vi "[ce low] Eval y=f(x).vi"(4 "include end point":bool, 5 "# points":u32=100, 6 "vm cmd":T1(ring), 7 "VC Handle":T2=-1, 8 "error in":errorcluster, 9 "formula info":cluster{"formula":string, "x-variable":string}={"formula"="", "x-variable"="t"}, 10 "end":dbl=1.0 format="%.2f", 11 "start":dbl format="%.2f") -> (0 "error out":errorcluster, 1 "dx":dbl format="%.2f", 2 "f(x)":dbl[](array[numeric]) format="%.2f", 3 "x":dbl[](array[numeric]) format="%.2f")   [LabVIEW 2021]
doc: "::: CalcExpress Toolkit :::\nCopyright (c) 2000-2026 Konstantin Shifershteyn. All rights reserved."
uses:
  cetypes.llb/VarMan Variable Context Handle.ctl
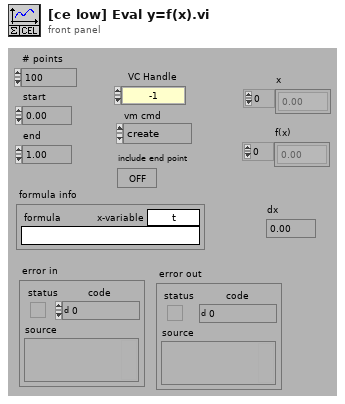
[diagram p1: front panel]
types:
  T1 = enum16{"create", "destroy", "set value", "get value"}
  T2 = typedef "VarMan Variable Context Handle.ctl" = i32
  T3 = typedef "VarMan Error Code.ctl" = u16
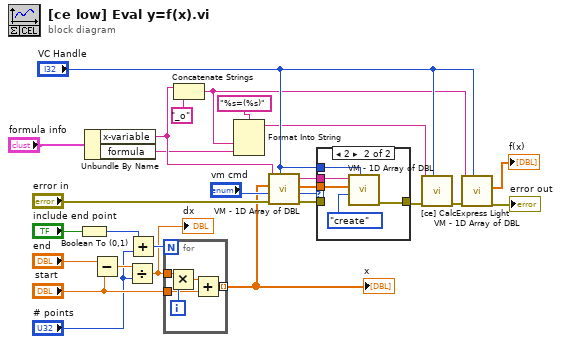
[diagram p0: block diagram]
diagram:
  n1 = Boolean To (0,1)(Boolean="include end point") -> (0, 1=w4:i16)
  n2 = Unbundle By Name("formula info") -> ("x-variable"=w18:string, "formula"=w13:string)
  n3 = Subtract(x="end", y="start") -> (x-y=w9:dbl)
  n4 = Divide(x=w9, y="# points") -> (x/y=w1:dbl)
  "dx" <- w1
  n5 = Add(x=w4, y="# points") -> (x+y=w3:u32)
  n6 = for {
    N: w3 -> [_]
    tunnel: w1 -> [w32]
    tunnel: "start" -> [w29]
    tunnel: [w28] -> w2 mode=indexing
    i -> [w31]
    n7 = Multiply(x=w32, y=w31) -> (x*y=w30:dbl)
    n8 = Add(x=w30, y=w29) -> (x+y=w28:dbl)
  }
  "x" <- w2
  n9 = Concatenate Strings(w18, "_o" ("Substring")) -> (w12:string)
  n10 = Format Into String(format string="%s=(%s)" ("Format String"), w12, w13) -> (resulting string=w11:string)  [unwired: 2 in, 1 out]
  n11 = call "VM - 1D Array of DBL.vi"("VC Handle"="VC Handle", "error in"="error in", "cmd"="vm cmd", "value in"=w2, "name_spec"=w18) -> ("error out"=w23:errorcluster, "err code"=w24:T3, "value out"=w22:dbl[], "dup name_spec"=w21:string)  [unwired: 1 in, 2 out]
  n12 = case shown="2" w24 {
    tunnel: w23 -> [w33 _]
    tunnel: [w33 w38] -> w20
    tunnel: w22 -> [_ w37]
    tunnel: w21 -> [_ w36]
    tunnel: "VC Handle" -> [_ w34]
    frame 0, Default {
    }
    frame 2 {
      n13 = call "VM - 1D Array of DBL.vi"("VC Handle"=w34, "cmd"=T1."create", "value in"=w37, "name_spec"=w36) -> ("error out"=w38:errorcluster)  [unwired: 2 in, 5 out]
    }
  }
  n14 = call "[ce] CalcExpress Light.vi"("VC Handle"="VC Handle", "error in"=w20, "expression"=w11) -> ("error out"=w26:errorcluster)  [unwired: 6 in, 2 out]
  n15 = call "VM - 1D Array of DBL.vi"("VC Handle"="VC Handle", "error in"=w26, "name_spec"=w12) -> ("error out"=→"error out":errorcluster, "value out"=→"f(x)":dbl[])  [unwired: 3 in, 4 out]
